vi "Lire config Th.vi"(2 "error in (no error)":errorcluster caption="entrée d'erreur (pas d'erreur)", 3 "refnum":T1) -> (0 "error out":errorcluster, 1 "refnum out":T1)   [LabVIEW 2022 SP3]
uses:
  <vilib>/Utility/config.llb/Config Data RefNum.ctl
  <vilib>/Utility/config.llb/Read Key (String).vi
  Variables globales/Variable glob Th.vi
  <vilib>/Utility/config.llb/Read Key (I32).vi
  <vilib>/Utility/config.llb/Read Key (Boolean).vi
  <vilib>/Utility/config.llb/NI_LVConfig.lvlib
panel:
  out "Nombre de chassis thermocouples":u8=1 min=1
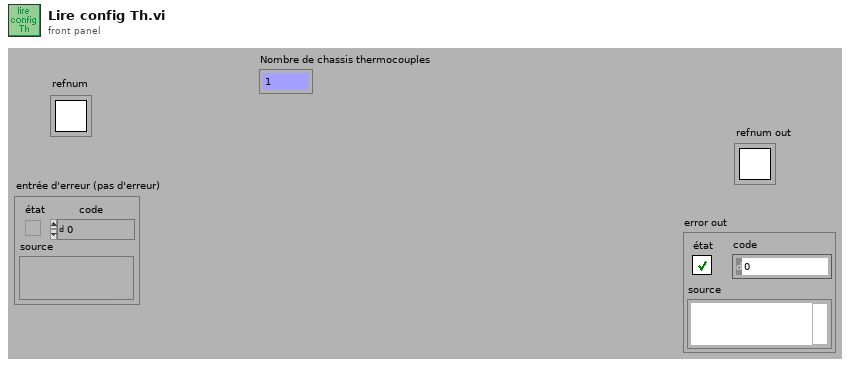
[diagram p1: front panel]
types:
  T1 = typedef "NI_LVConfig.lvlib/Config Data RefNum.ctl" = refnum<k1>
  T2 = cluster{"Nom tache Th":refnum<k21>, "Noms des Th":string[], "Nb Th":i16, "Sélection Th":bool[], "Nom Th sélectionnées":string[]}[]
  T3 = cluster{"Nom tache Th":refnum<k21>, "Noms des Th":string[], "Nb Th":i16, "Selection Th":bool[], "Nom Th selectionnes":string[]}[]
  T4 = cluster{"Nom tache Th":refnum<k21>, "Noms des Th":string[], "Nb Th":i16, "Selection Th":bool[], "Nom Th selectionnes":string[]}
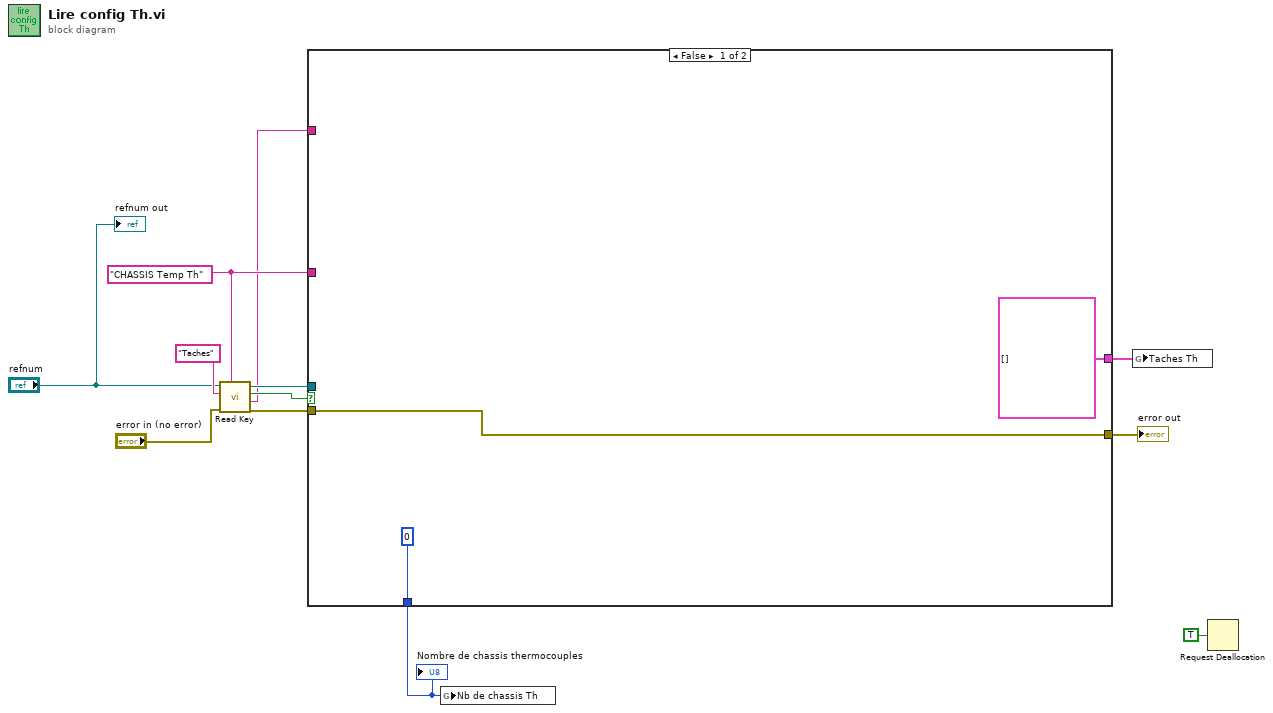
[diagram p0: block diagram]
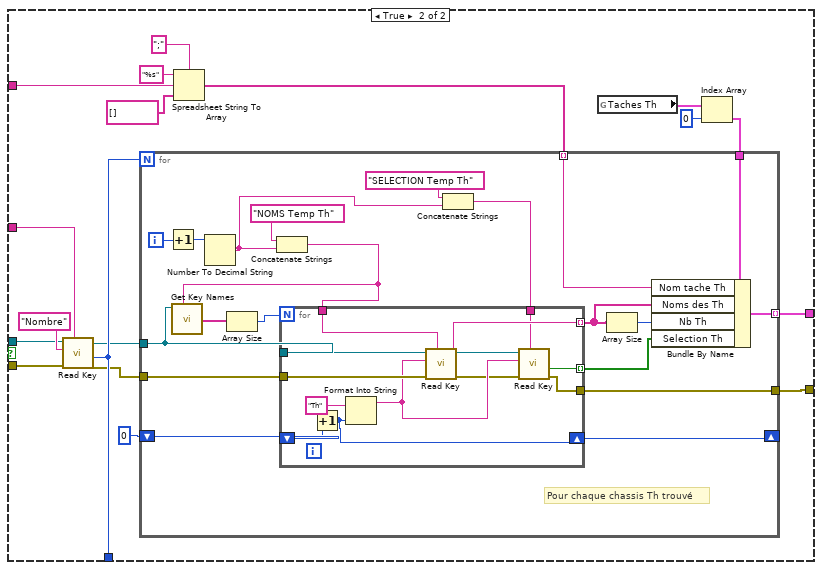
[diagram p2: hidden frame]
diagram:
  w11 = "CHASSIS Temp Th" ("section")
  n1 = call-poly <vilib>:"Read Key.vi"("section"=w11, "error in (no error)"="error in (no error)", "key"="Taches", "refnum"="refnum") -> ("error out"=w8:errorcluster, "value"=w1:string, "found?"=w5:bool, "refnum out"=w7:T1)  [unwired: 4 in]
  n2 = case shown="False" w5 {
    tunnel: [0 ("value") w33] -> w12
    tunnel: w11 -> [_ w29]
    tunnel: [w14 w32] -> w10
    tunnel: w8 -> [w14 w27]
    tunnel: w7 -> [_ w28]
    tunnel: [T2 [] w16] -> w4
    tunnel: w1 -> [_ w21]
    frame False {
    }
    frame True {
      n3 = call-poly <vilib>:"Read Key.vi"("section"=w29, "error in (no error)"=w27, "key"="Nombre", "refnum"=w28) -> ("error out"=w25:errorcluster, "value"=w33:i32, "refnum out"=w26:T1)  [unwired: 4 in, 1 out]
      n4 = Spreadsheet String To Array(delimiter (Tab)=";" ("séparateur (Tabulation)"), format string="%s" ("chaîne de format"), spreadsheet string=w21, array type (2D Dbl)=string[] [] ("type de tableau (2D de dbl)")) -> (array=w17:string[])
      n5 = global read "Variable glob Th.vi" "Taches Th"() -> (w20:T3)
      n6 = Index Array(array=w20, index=0 ("indice")) -> (element=w18:T4)
      n7 = for {
        N: w33 -> [_]
        tunnel: [w53] -> w32
        tunnel: w26 -> [w43]
        tunnel: w25 -> [w52]
        shift-right: [w48] -> _
        shift-left: 0 -> [w49]
        tunnel: w18 -> [w39]
        tunnel: w17 -> [w38] mode=indexing
        tunnel: [w34] -> w16 mode=indexing
        i -> [w51]
        # "Pour chaque chassis Th trouvé"
        n8 = Increment(x=w51) -> (x+1=w50:i32)
        n9 = Number To Decimal String(number=w50) -> (decimal integer string=w40:string)  [unwired: 1 in]
        n10 = Concatenate Strings("NOMS Temp Th" ("chaîne initiale"), w40) -> (w44:string)
        n11 = call <vilib>:"Get Key Names.vi"("section"=w44, "refnum"=w43) -> ("key names"=w42:string[])  [unwired: 6 in, 3 out]
        n12 = Array Size(array=w42) -> (size(s)=w41:i32)
        n13 = Concatenate Strings("SELECTION Temp Th" ("chaîne initiale"), w40) -> (w45:string)
        n14 = for {
          N: w41 -> [_]
          tunnel: w43 -> [w66]
          tunnel: w52 -> [w65]
          tunnel: [w61] -> w37 mode=indexing
          tunnel: [w63] -> w35 mode=indexing
          tunnel: [w62] -> w53
          shift-right: [w59] -> w48
          shift-left: w49 -> [w60]
          tunnel: w45 -> [w58]
          tunnel: w44 -> [w57]
          n15 = Increment(x=w60) -> (x+1=w59:i32)
          n16 = Format Into String(initial string="Th" ("chaîne initiale"), w59) -> (resulting string=w56:string)  [unwired: 2 in, 1 out]
          n17 = call-poly <vilib>:"Read Key.vi"("section"=w57, "error in (no error)"=w65, "key"=w56, "refnum"=w66) -> ("error out"=w54:errorcluster, "value"=w61:string, "refnum out"=w55:T1)  [unwired: 4 in, 1 out]
          n18 = call-poly <vilib>:"Read Key.vi"("section"=w58, "error in (no error)"=w54, "key"=w56, "refnum"=w55) -> ("error out"=w62:errorcluster, "value"=w63:bool)  [unwired: 4 in, 2 out]
        }
        n19 = Array Size(array=w37) -> (size(s)=w36:i32)
        n20 = Bundle By Name(cluster=w39, "Nom tache Th"=w38, "Noms des Th"=w37, "Nb Th"=w36, "Selection Th"=w35) -> (w34:T4)
      }
    }
  }
  "Nombre de chassis thermocouples" <- w12
  "error out" <- w10
  n21 = global write "Variable glob Th.vi" "Nb de chassis Th"(w12) -> ()
  n22 = global write "Variable glob Th.vi" "Taches Th"(w4) -> ()
  n23 = Request Deallocation(TRUE ("flag")) -> ()
  "refnum out" <- "refnum"
